vi "Abort Status Check.vi"(8 "error in (no error)":errorcluster, 11 "Guardian in":refnum<class "Guardian.lvclass">) -> (0 "error out":errorcluster, 3 "Guardian out":refnum<class "Guardian.lvclass">)   [LabVIEW 2020, in "TALOS.lvlib" / "Guardian.lvlib" / "Guardian.lvclass"]
doc: "This VI is called periodically to check the health status of ABORT and its unicity."
uses:
  Guardian.lvclass
  C:/Users/marco/Documents/GitHub_Lab/TALOS/talos/Ancestor/Ancestor/Ancestor.lvclass
  C:/Users/marco/Documents/GitHub_Lab/TALOS/builds/Actor Framework PPL/Actor Framework.lvlibp/1abvi3w/vi.lib/ActorFramework/Actor/Actor.lvclass
  Guardian.lvclass/Guardian.ctl
  Ancestor/Ancestor/Ancestor.lvclass/Ancestor.ctl
  Classes/Speedometer/Speedometer.lvclass/Speedometer.ctl
  Guardian Messages/Message to Other Guardian Msg/Message to Other Guardian Msg.lvclass/Message to Other Guardian Msg.ctl
  Guardian Messages/TCP-SV Message Interpreter Msg/TCP-SV Message Interpreter Msg.lvclass/TCP-SV Message Interpreter Msg.ctl
  4755b682-1248-473b-8cd2-dfaaffe09b65.vi
  cbc8a120-93e6-4d44-b253-7cefa591677c.vi
  3ae19a6a-4145-421c-a6fa-2879faec311c.vi
  Support VIs/Generate Error.vi
  <vilib>/Utility/High Resolution Relative Seconds.vi
  Broadcast to Guardians.vi
  FGV/Error Memory/Get Error Description.vi
  Support VIs/Get PC name.vi
  Support VIs/Get Class Name.vi
  Guardian Messages/Message to Other Guardian Msg/Send Message to Other Guardian.vi
  Support VIs/Search Array of Strings.vi
  Guardian Messages/TCP-SV Message Interpreter Msg/Send TCP-SV Message Interpreter.vi
  FGV/Error Memory/Error Memory Core.vi
  <vilib>/AdvancedString/Delimited String to 1D String Array.vi
  Support VIs/Circus Root Path.vi
  FGV/Error Memory/Error Crt Lvl checker.vi
  FGV/Error Memory/Error Memory Core.vi/40c8088d-b597-4017-91af-faa98e00292e.vi
  FGV/Error Memory/Error Memory Core.vi/d4a3ab98-063c-4e44-b43d-fbdcfe6c2be2.vi
  Support VIs/Global Memory.vi
  <vilib>/Utility/LVClass/Get LV Class Name.vi
  Support VIs/Is in Packed Library.vi
  Support VIs/TALOS Root path.vi
  Support VIs/Read CSV worksheet.vi
  Support VIs/Global Constants.vi
  <vilib>/Utility/error.llb/General Error Handler.vi
  <vilib>/Utility/config.llb/Open Config Data.vi
  <vilib>/Utility/config.llb/Get Section Names.vi
  <vilib>/Utility/config.llb/Get Key Names.vi
  <vilib>/Utility/config.llb/Read Key.vi
  <vilib>/Utility/config.llb/Read Key (String).vi
  <vilib>/Utility/config.llb/Close Config Data.vi
  Pat message.vi
  Support VIs/Circus Critical PCs List.vi
  builds/Actor Framework PPL/Actor Framework.lvlibp/1abvi3w/vi.lib/ActorFramework/Actor/Read Self Enqueuer.vi
  builds/Actor Framework PPL/Actor Framework.lvlibp/1abvi3w/vi.lib/ActorFramework/Message Enqueuer/Enqueue.vi
  Support VIs/Error Log.vi
  Support VIs/System Log.vi
  Ancestor/Ancestor/Ancestor.lvclass
  <vilib>/Comparison/Equal/Equal Functor/Equal Functor.lvclass
  Classes/Speedometer/Speedometer.lvclass
  <vilib>/Comparison/Less/Less Functor/Less Functor.lvclass
  Guardian Messages/Message to Other Guardian Msg/Message to Other Guardian Msg.lvclass
  Guardian Messages/TCP-SV Message Interpreter Msg/TCP-SV Message Interpreter Msg.lvclass
  Classes/Guardian List/Guardian List.lvclass
  TALOS.lvlib
  C:/Users/marco/Documents/GitHub_Lab/TALOS/talos/Guardian/Guardian/Guardian.lvclass
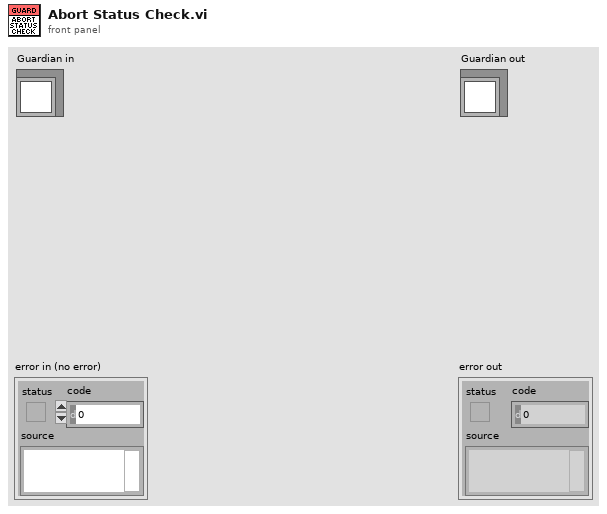
[diagram p1: front panel]
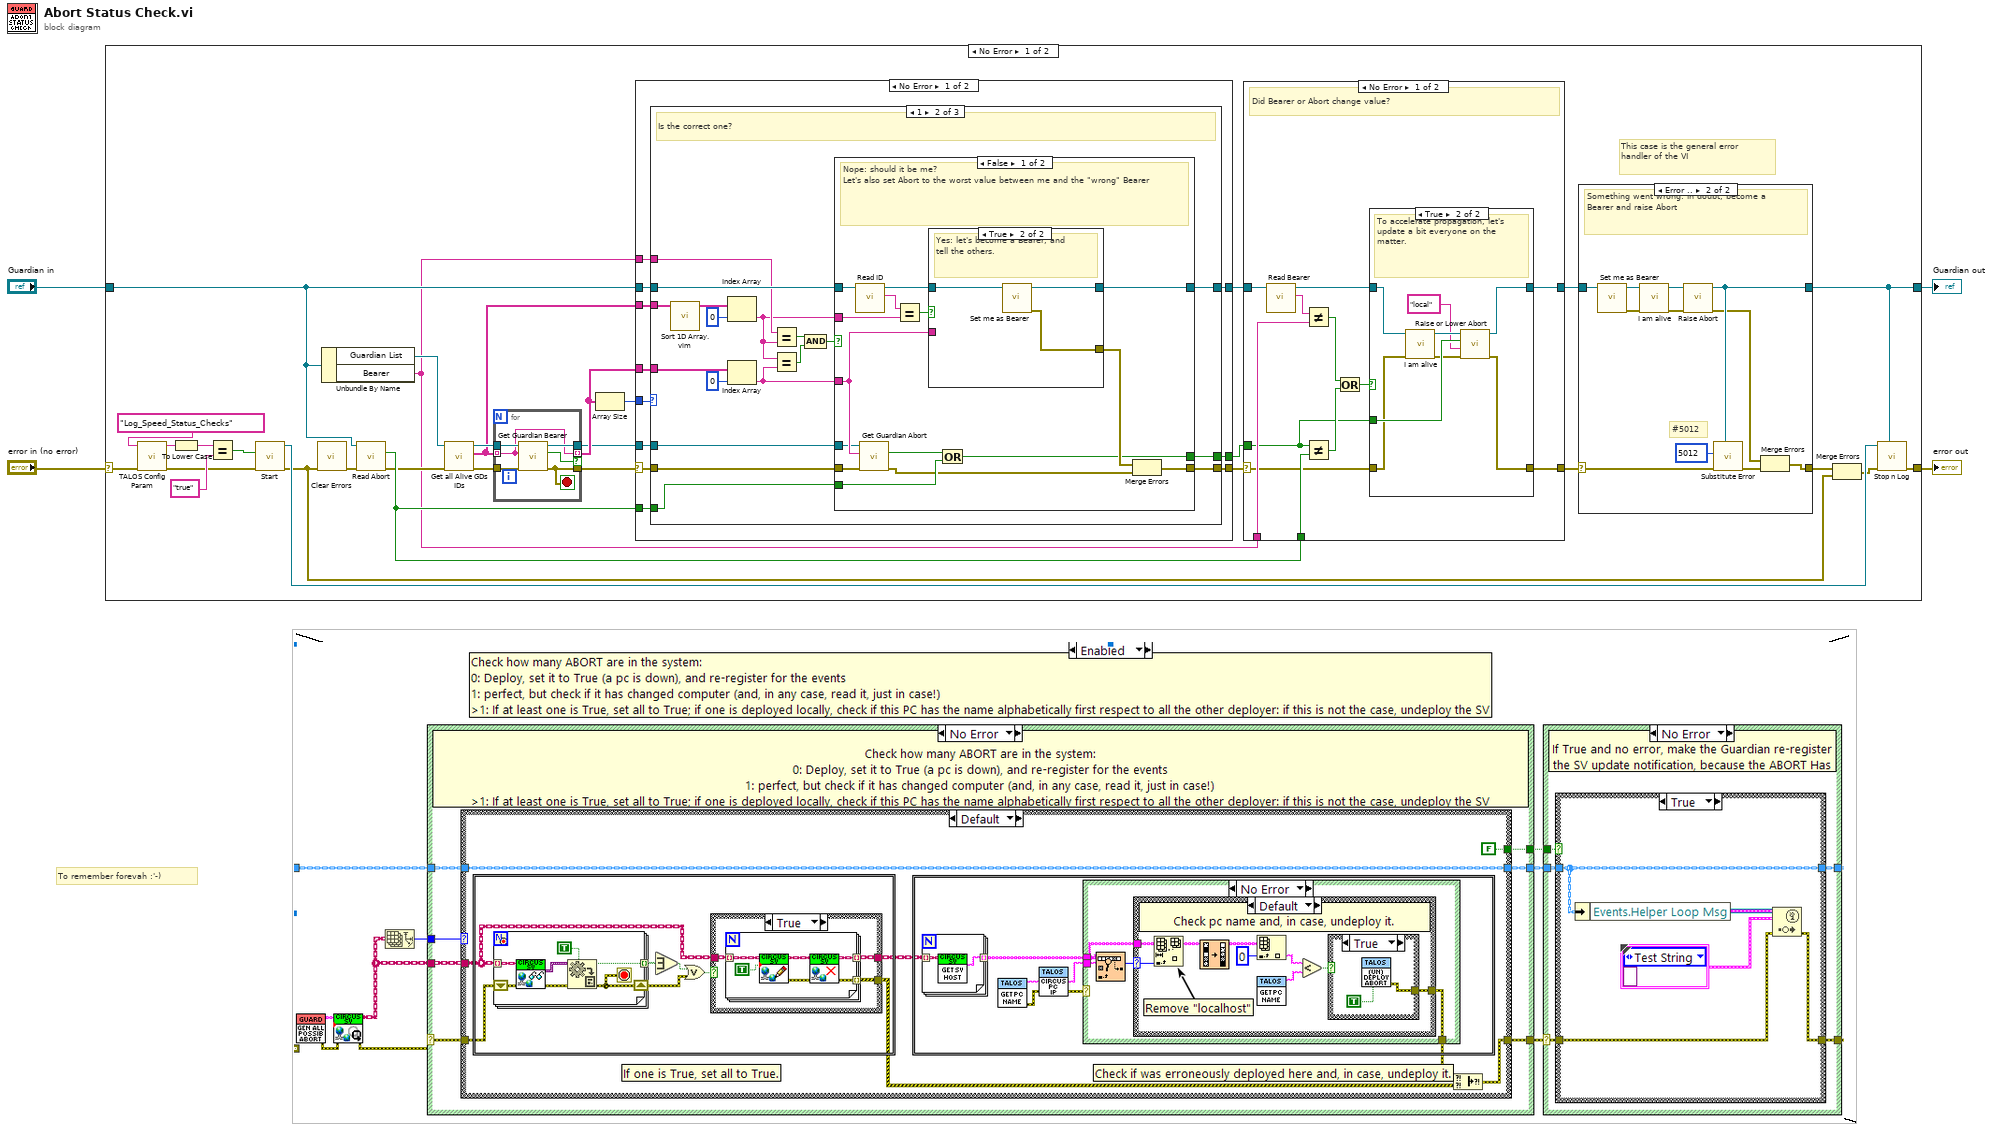
[diagram p0: block diagram]
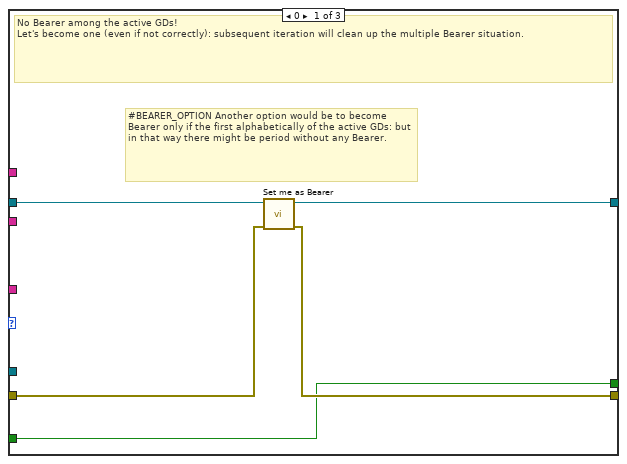
[diagram p4: hidden frame]
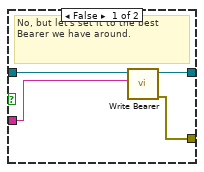
[diagram p5: hidden frame]
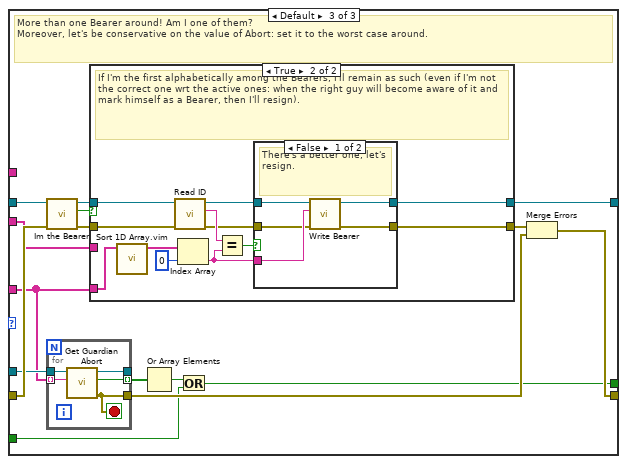
[diagram p7: hidden frame]
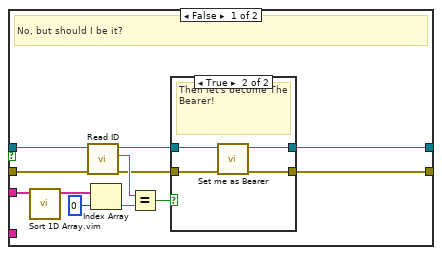
[diagram p8: hidden frame]
diagram:
  # "To remember forevah :'-)"
  n1 = case shown="No Error" "error in (no error)" {
    selector: "error in (no error)" -> [w25 w200]
    tunnel: [w34 w199] -> w1
    tunnel: [w33 w200] -> w3
    tunnel: "Guardian in" -> [w6 w199]
    frame No Error {
      # "This case is the general error handler of the VI"
      n2 = call "TALOS Config Param.vi"("error in (no error)"=w25, "Parameter Name"="Log_Speed_Status_Checks") -> ("error out"=w27:errorcluster, "Output"=w32:string)  [unwired: 8 in]
      n3 = To Lower Case(string=w32) -> (all lower case string=w31:string)
      n4 = Equal?(x=w31, y="true") -> (x = y?=w28:bool)
      n5 = call "Start.vi"("error in (no error)"=w27, "Active?"=w28) -> ("error out"=w23:errorcluster, "Speedometer out"=w35:refnum<class "Speedometer.lvclass">)  [unwired: 8 in]
      n6 = call <vilib>:"Clear Errors.vi"("error in (no error)"=w23) -> ("error out"=w9:errorcluster)  [unwired: 5 in, 1 out]
      n7 = Unbundle By Name(w6) -> ("Guardian List"=w20:refnum<class "Guardian List.lvclass">, "Bearer"=w5:string)
      n8 = call "Read Abort.vi"("error in (no error)"=w9, "Guardian in"=w6) -> ("error out"=w7:errorcluster, "Abort"=w8:bool)  [unwired: 7 in, 1 out]
      n9 = call-dynamic "Get all Alive GDs IDs.vi"("error in (no error)"=w7, "Guardian List in"=w20) -> ("error out"=w18:errorcluster, "Alive GDs IDs"=w15:string[], "Guardian List out"=w19:refnum<class "Guardian List.lvclass">)  [unwired: 7 in]
      n10 = for {
        tunnel: w19 -> [w184]
        tunnel: w15 -> [w181] mode=indexing
        tunnel: w18 -> [w185]
        tunnel: [w183] -> w13
        tunnel: [w182] -> w16
        tunnel: [w181] -> w14 mode=indexing if=w180
        stop <- w182 stop-if-true
        n11 = call-dynamic "Get Guardian Bearer.vi"("error in (no error)"=w185, "ID"=w181, "Guardian List in"=w184) -> ("error out"=w182:errorcluster, "Bearer"=w180:bool, "Guardian List out"=w183:refnum<class "Guardian List.lvclass">)  [unwired: 6 in]
      }
      n12 = Array Size(array=w14) -> (size(s)=w17:i32)
      n13 = case shown="No Error" w16 {
        selector: w16 -> [w69 w178]
        tunnel: w17 -> [w70 _]
        tunnel: w15 -> [w68 _]
        tunnel: w14 -> [w67 _]
        tunnel: w6 -> [w66 w179]
        tunnel: [w65 w179] -> w22
        tunnel: [w64 w178] -> w21
        tunnel: w13 -> [w63 _]
        tunnel: w8 -> [w62 w177]
        tunnel: [w61 w177] -> w10
        tunnel: w5 -> [w60 _]
        frame No Error {
          n14 = case shown="1" w70 {
            tunnel: w69 -> [w72 w87 w132]
            tunnel: w68 -> [_ w93 w126]
            tunnel: w67 -> [_ w89 w125]
            tunnel: w66 -> [w73 w86 w133]
            tunnel: [w75 w85 w122] -> w65
            tunnel: [w74 w84 w120] -> w64
            tunnel: w63 -> [_ w83 w128]
            tunnel: w62 -> [w71 w82 w123]
            tunnel: [w71 w81 w119] -> w61
            tunnel: w60 -> [_ w80 _]
            frame 0 {
              # "#BEARER_OPTION Another option would be to become Bearer only if the first alphabetically of the active GDs: but in that way there might be period without any Bearer."
              # "No Bearer among the active GDs!\nLet's become one (even if not correctly): subsequent iteration will clean up the multiple Bearer situation."
              n15 = call "Set me as Bearer.vi"("error in"=w72, "Guardian in"=w73) -> ("error out"=w74:errorcluster, "Guardian out"=w75:refnum<class "Guardian.lvclass">)  [unwired: 8 in]
            }
            frame 1 {
              # "Is the correct one?"
              n16 = call "Sort 1D Array.vim"("unsorted array"=w93) -> ("sorted array"=w92:string[])  [unwired: 10 in]
              n17 = Index Array(array=w92, index=0) -> (element=w77:string)
              n18 = Index Array(array=w89, index=0) -> (element=w78:string)
              n19 = Equal?(x=w80, y=w77) -> (x = y?=w88:bool)
              n20 = Equal?(x=w77, y=w78) -> (x = y?=w76:bool)
              n21 = And(x=w88, y=w76) -> (x .and. y?=w79:bool)
              n22 = case shown="False" w79 {
                tunnel: w87 -> [w103 w117]
                tunnel: w86 -> [w108 w118]
                tunnel: w77 -> [w107 _]
                tunnel: [w102 w118] -> w85
                tunnel: [w95 w117] -> w84
                tunnel: w78 -> [w100 _]
                tunnel: w83 -> [w97 _]
                tunnel: w82 -> [w99 w116]
                tunnel: [w96 w116] -> w81
                frame False {
                  # "Nope: should it be me?\nLet's also set Abort to the worst value between me and the \"wrong\" Bearer"
                  n23 = call "Read ID.vi"("Ancestor in"=w108) -> ("ID"=w104:string, "Ancestor out"=w105:refnum<class "Guardian.lvclass">)  [unwired: 8 in, 1 out]
                  n24 = call-dynamic "Get Guardian Abort.vi"("error in (no error)"=w103, "ID"=w100, "Guardian List in"=w97) -> ("error out"=w94:errorcluster, "Abort"=w98:bool)  [unwired: 6 in, 1 out]
                  n25 = Equal?(x=w104, y=w107) -> (x = y?=w106:bool)
                  n26 = case shown="True" w106 {
                    tunnel: w105 -> [w112 w115]
                    tunnel: [w111 w114] -> w102
                    tunnel: [w109 w113] -> w101
                    tunnel: w100 -> [w110 _]
                    frame False {
                      # "No, but let's set it to the best Bearer we have around."
                      n27 = call "Write Bearer.vi"("Bearer"=w110, "Guardian in"=w112) -> ("error out"=w109:errorcluster, "Guardian out"=w111:refnum<class "Guardian.lvclass">)  [unwired: 8 in]
                    }
                    frame True {
                      # "Yes: let's become a Bearer, and tell the others."
                      n28 = call "Set me as Bearer.vi"("Guardian in"=w115) -> ("error out"=w113:errorcluster, "Guardian out"=w114:refnum<class "Guardian.lvclass">)  [unwired: 9 in]
                    }
                  }
                  n29 = Or(x=w98, y=w99) -> (x .or. y?=w96:bool)
                  n30 = Merge Errors(w101, w94) -> (w95:errorcluster)
                }
                frame True {
                  # "Perfect, all good."
                }
              }
            }
            frame Default {
              # "More than one Bearer around! Am I one of them?\nMoreover, let's be conservative on the value of Abort: set it to the worst case around."
              n31 = call "Im the Bearer.vi"("error in (no error)"=w132, "Guardian in"=w133) -> ("error out"=w131:errorcluster, "I'm the Bearer"=w130:bool, "Guardian out"=w129:refnum<class "Guardian.lvclass">)  [unwired: 7 in]
              n32 = for {
                tunnel: w128 -> [w139]
                tunnel: w125 -> [w138] mode=indexing
                tunnel: [w137] -> _
                tunnel: [w136] -> w127 mode=indexing
                tunnel: [w135] -> w134
                stop <- w135 stop-if-true
                n33 = call-dynamic "Get Guardian Abort.vi"("ID"=w138, "Guardian List in"=w139) -> ("error out"=w135:errorcluster, "Abort"=w136:bool, "Guardian List out"=w137:refnum<class "Guardian List.lvclass">)  [unwired: 7 in]
              }
              n34 = case shown="True" w130 {
                tunnel: w131 -> [w145 w165]
                tunnel: w129 -> [w147 w166]
                tunnel: w126 -> [w148 _]
                tunnel: w125 -> [_ w164]
                tunnel: [w141 w159] -> w122
                tunnel: [w140 w158] -> w121
                frame False {
                  # "No, but should I be it?"
                  n35 = call "Sort 1D Array.vim"("unsorted array"=w148) -> ("sorted array"=w151:string[])  [unwired: 10 in]
                  n36 = call "Read ID.vi"("error in (no error)"=w145, "Ancestor in"=w147) -> ("error out"=w143:errorcluster, "ID"=w149:string, "Ancestor out"=w142:refnum<class "Guardian.lvclass">)  [unwired: 7 in]
                  n37 = Index Array(array=w151, index=0) -> (element=w146:string)
                  n38 = Equal?(x=w149, y=w146) -> (x = y?=w144:bool)
                  n39 = case shown="True" w144 {
                    tunnel: w143 -> [w152 w156]
                    tunnel: w142 -> [w153 w157]
                    tunnel: [w153 w155] -> w141
                    tunnel: [w152 w154] -> w140
                    frame False {
                      # "Nope, let's relax."
                    }
                    frame True {
                      # "Then let's become The Bearer!"
                      n40 = call "Set me as Bearer.vi"("error in"=w156, "Guardian in"=w157) -> ("error out"=w154:errorcluster, "Guardian out"=w155:refnum<class "Guardian.lvclass">)  [unwired: 8 in]
                    }
                  }
                }
                frame True {
                  # "If I'm the first alphabetically among the Bearers, I'll remain as such (even if I'm not the correct one wrt the active ones: when the right guy will become aware of it and mark himself as a Bearer, then I'll resign)."
                  n41 = call "Sort 1D Array.vim"("unsorted array"=w164) -> ("sorted array"=w169:string[])  [unwired: 10 in]
                  n42 = call "Read ID.vi"("error in (no error)"=w165, "Ancestor in"=w166) -> ("error out"=w161:errorcluster, "ID"=w167:string, "Ancestor out"=w162:refnum<class "Guardian.lvclass">)  [unwired: 7 in]
                  n43 = Index Array(array=w169, index=0) -> (element=w160:string)
                  n44 = Equal?(x=w167, y=w160) -> (x = y?=w163:bool)
                  n45 = case shown="False" w163 {
                    tunnel: w162 -> [w174 w176]
                    tunnel: w161 -> [w172 w175]
                    tunnel: w160 -> [w173 _]
                    tunnel: [w171 w176] -> w159
                    tunnel: [w170 w175] -> w158
                    frame False {
                      # "There's a better one, let's resign."
                      n46 = call "Write Bearer.vi"("error in (no error)"=w172, "Bearer"=w173, "Guardian in"=w174) -> ("error out"=w170:errorcluster, "Guardian out"=w171:refnum<class "Guardian.lvclass">)  [unwired: 7 in]
                    }
                    frame True {
                      # "\"Most correct\" one possible."
                    }
                  }
                }
              }
              n47 = Or Array Elements(Boolean array=w127) -> (logical OR=w124:bool)
              n48 = Or(x=w124, y=w123) -> (x .or. y?=w119:bool)
              n49 = Merge Errors(w121, w134) -> (w120:errorcluster)
            }
          }
        }
        frame Error {
          # "It should never happen, but you know..."
        }
      }
      n50 = case shown="No Error" w21 {
        selector: w21 -> [w36 w58]
        tunnel: w22 -> [w47 w59]
        tunnel: w5 -> [w46 _]
        tunnel: w8 -> [w41 _]
        tunnel: [w39 w59] -> w12
        tunnel: [w38 w58] -> w11
        tunnel: w10 -> [w37 _]
        frame No Error {
          # "Did Bearer or Abort change value?"
          n51 = call "Read Bearer.vi"("Guardian in"=w47) -> ("Bearer"=w45:string, "Guardian out"=w40:refnum<class "Guardian.lvclass">)  [unwired: 8 in, 1 out]
          n52 = Not Equal?(x=w45, y=w46) -> (x != y?=w44:bool)
          n53 = Not Equal?(x=w37, y=w41) -> (x != y?=w43:bool)
          n54 = Or(x=w44, y=w43) -> (x .or. y?=w42:bool)
          n55 = case shown="True" w42 {
            tunnel: w36 -> [w48 w54]
            tunnel: w40 -> [w49 w57]
            tunnel: [w49 w51] -> w39
            tunnel: [w48 w52] -> w38
            tunnel: w37 -> [_ w56]
            frame False {
              # "Nothing changed, do nothing."
            }
            frame True {
              # "To accelerate propagation, let's update a bit everyone on the matter."
              n56 = call "I am alive.vi"("error in (no error)"=w54, "Guardian in"=w57) -> ("error out"=w53:errorcluster, "Guardian out"=w55:refnum<class "Guardian.lvclass">)  [unwired: 8 in]
              n57 = call "Raise or Lower Abort.vi"("error in (no error)"=w53, "Sender"="local", "New Abort Value"=w56, "Guardian in"=w55) -> ("error out"=w52:errorcluster, "Guardian out"=w51:refnum<class "Guardian.lvclass">)  [unwired: 6 in]
            }
          }
        }
        frame Error {
          # "An error occurred, just go to the error handling of this VI."
        }
      }
      n58 = case shown="Error .." w11 {
        selector: w11 -> [w187 w193]
        tunnel: [w186 w192] -> w34
        tunnel: [w187 w189] -> w26
        tunnel: w12 -> [w186 w188]
        frame No Error {
          # "All good!"
        }
        frame Error {
          # "#5012"
          # "Something went wrong: in doubt, become a Bearer and raise Abort"
          n59 = call "Set me as Bearer.vi"("Guardian in"=w188) -> ("error out"=w195:errorcluster, "Guardian out"=w196:refnum<class "Guardian.lvclass">)  [unwired: 9 in]
          n60 = call "I am alive.vi"("error in (no error)"=w195, "Guardian in"=w196) -> ("error out"=w198:errorcluster, "Guardian out"=w197:refnum<class "Guardian.lvclass">)  [unwired: 8 in]
          n61 = call "Raise Abort.vi"("error in (no error)"=w198, "Guardian in"=w197) -> ("error out"=w191:errorcluster, "Guardian out"=w192:refnum<class "Guardian.lvclass">)  [unwired: 8 in]
          n62 = call "Substitute Error.vi"("LabVIEW Object"=w192, "error in (no error)"=w193, "Error Code"=5012) -> ("error out"=w190:errorcluster)  [unwired: 8 in]
          n63 = Merge Errors(w191, w190) -> (w189:errorcluster)
        }
      }
      n64 = Merge Errors(w26, w23) -> (w24:errorcluster)
      n65 = call "Stop n Log.vi"("Object in"=w34, "error in (no error)"=w24, "Speedometer in"=w35) -> ("error out"=w33:errorcluster)  [unwired: 8 in]
    }
    frame Error {
    }
  }
  "error out" <- w3
  "Guardian out" <- w1
